vi "Bench Encode PNG.vi"() -> ()   [LabVIEW 2020]
doc: "Benchmark for RemoteVI Capture Panel.vi and RemoteVI Encode Rect PNG.vi. Opens the panel of the VI at VI Path, waits, captures it once (timed), closes the panel and the reference without saving, then encodes the full capture and a 64-row band at every compression level in Levels and reports the average milliseconds and PNG sizes. Writes the full capture, encoded with the default compression, to PNG Path."
uses:
  source/RemoteVI.lvlib
panel:
  out "error out":errorcluster
  out "default png bytes":i32
  out "band bytes":i32[](array[numeric])
  out "band ms":dbl[](array[numeric])
  out "full bytes":i32[](array[numeric])
  out "full ms":dbl[](array[numeric])
  out "capture ms":i32
  out "height":i32
  out "width":i32
  in  "Settle ms":i32=1000
  in  "Band Top":i32=256
  in  "Band Reps":i32=20
  in  "Full Reps":i32=5
  in  "Levels":i32[](array[numeric])=[0, 1, 2, 3, 6, 9]
  in  "PNG Path":path=path "C:/Users/jgoebel/OneDrive - Emerson/Dokumente/git_repos/RemoteVI/spikes/encode_check.png"
  in  "VI Path":path=path "C:/Program Files/National Instruments/LabVIEW 2025/examples/Controls and Indicators/Containers/Resizable Panel with Splitter Bars.vi"
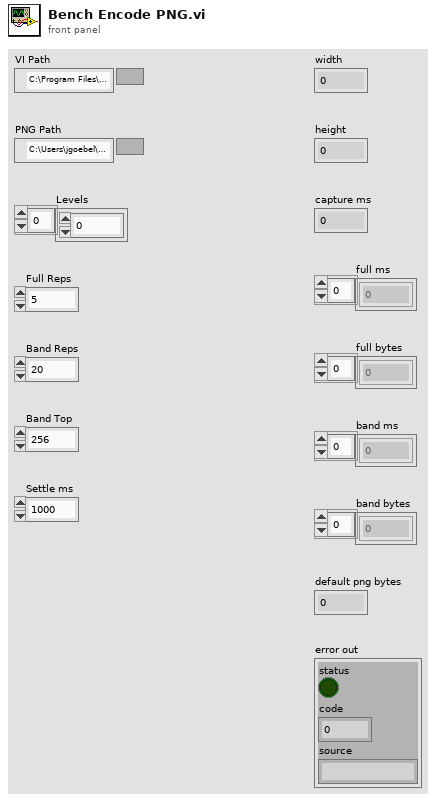
[diagram p1: front panel]
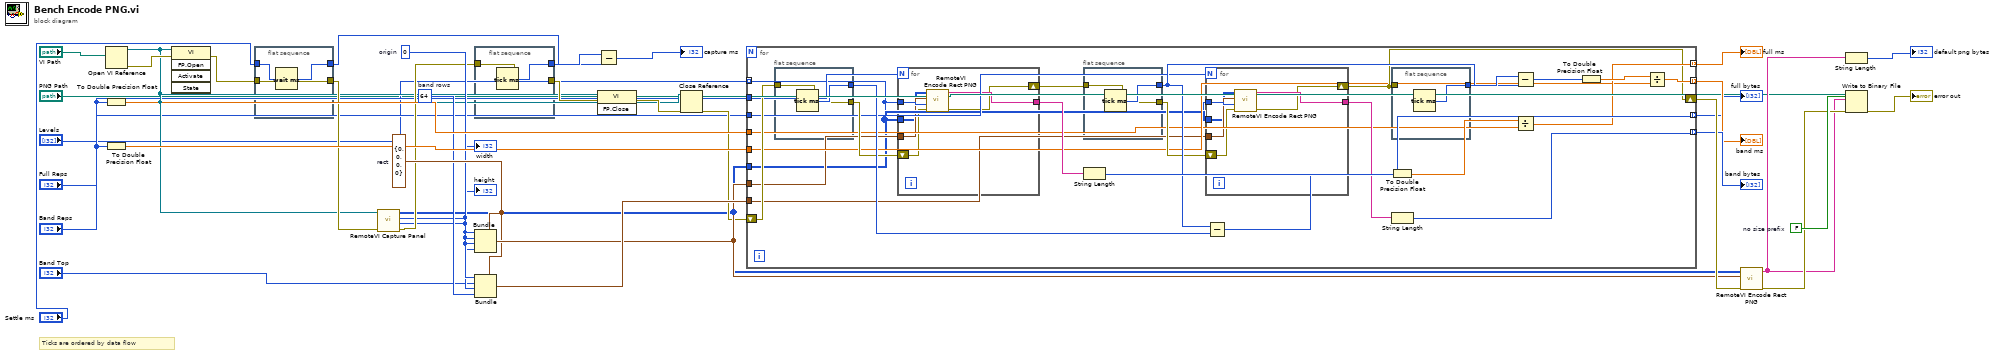
[diagram p0: block diagram]
diagram:
  w38 = FALSE  # no size prefix
  w30 = cluster{"x":i32, "y":i32, "w":i32, "h":i32} {"x"=0, "y"=0, "w"=0, "h"=0}  # rect
  w29 = 64  # band rows
  w28 = 0  # origin
  # "Ticks are ordered by data flow"
  n1 = Open VI Reference(vi path="VI Path") -> (vi reference=w17:refnum<vi>, error out=w18:errorcluster)  [unwired: 5 in]
  n2 = To Double Precision Float(number="Full Reps") -> (double precision float=w33:dbl)
  n3 = To Double Precision Float(number="Band Reps") -> (double precision float=w34:dbl)
  n4 = invoke class="VI" method="FP.Open"(reference=w17, error in=w18) -> (error out=w19:errorcluster)  [unwired: 3 in, 4 out]
  n5 = flat-sequence {
    tunnel: "Settle ms" -> [w40]
    tunnel: w19 -> [w39]
    tunnel: [w41] -> w21
    tunnel: [w39] -> w20
    frame #0 {
      n6 = Wait (ms)(milliseconds to wait=w40) -> (millisecond timer value=w41:i32)
    }
  }
  n7 = call "RemoteVI Capture Panel.vi"("error in"=w20, "VI"=w17) -> ("error out"=w23:errorcluster, "height"=w9:i32, "width"=w8:i32, "pixmap"=w22:u32[][])  [unwired: 6 in]
  "width" <- w8
  "height" <- w9
  n8 = flat-sequence {
    tunnel: [w43] -> w25
    tunnel: w23 -> [w42]
    tunnel: [w42] -> w24
    frame #0 {
      n9 = Tick Count (ms)() -> (millisecond timer value=w43:u32)
    }
  }
  n10 = Bundle(cluster=w30, "x"=w28, "y"=w28, "w"=w8, "h"=w9) -> (w31:cluster{"x":i32, "y":i32, "w":i32, "h":i32})
  n11 = Bundle(cluster=w30, "x"=w28, "y"="Band Top", "w"=w8, "h"=w29) -> (w32:cluster{"x":i32, "y":i32, "w":i32, "h":i32})
  n12 = Subtract(x=w25, y=w21) -> (x-y=→"capture ms":u32)
  n13 = invoke class="VI" method="FP.Close"(reference=w17, error in=w24) -> (error out=w26:errorcluster)  [unwired: 1 in, 2 out]
  n14 = Close Reference(reference=w17, error in (no error)=w26) -> (error out=w27:errorcluster)
  n15 = for {
    tunnel: "Levels" -> [w44] mode=indexing
    tunnel: "Full Reps" -> [w48]
    tunnel: "Band Reps" -> [w49]
    tunnel: w33 -> [w50]
    tunnel: w34 -> [w51]
    tunnel: w22 -> [w45]
    tunnel: [w64] -> w11 mode=indexing
    tunnel: [w67] -> w13 mode=indexing
    tunnel: w31 -> [w46]
    tunnel: w32 -> [w47]
    shift-right: [w53] -> w35
    shift-left: w27 -> [w52]
    tunnel: [w68] -> w12 mode=indexing
    tunnel: [w69] -> w14 mode=indexing
    n16 = flat-sequence {
      tunnel: [w86] -> w55
      tunnel: w52 -> [w85]
      tunnel: [w85] -> w54
      frame #0 {
        n17 = Tick Count (ms)() -> (millisecond timer value=w86:u32)
      }
    }
    n18 = for {
      N: w48 -> [_]
      tunnel: w44 -> [w81]
      tunnel: w45 -> [w79]
      tunnel: w46 -> [w80]
      shift-right: [w83] -> w56
      shift-left: w54 -> [w82]
      tunnel: [w84] -> w57
      n19 = call "RemoteVI Encode Rect PNG.vi"("error in"=w82, "compression"=w81, "rect"=w80, "pixmap"=w79) -> ("error out"=w83:errorcluster, "png"=w84:string)  [unwired: 6 in]
    }
    n20 = flat-sequence {
      tunnel: [w78] -> w59
      tunnel: w56 -> [w77]
      tunnel: [w77] -> w58
      frame #0 {
        n21 = Tick Count (ms)() -> (millisecond timer value=w78:u32)
      }
    }
    n22 = String Length(string=w57) -> (length=w68:i32)
    n23 = for {
      N: w49 -> [_]
      tunnel: w44 -> [w73]
      tunnel: w45 -> [w71]
      tunnel: w47 -> [w72]
      shift-right: [w75] -> w53
      shift-left: w58 -> [w74]
      tunnel: [w76] -> w60
      n24 = call "RemoteVI Encode Rect PNG.vi"("error in"=w74, "compression"=w73, "rect"=w72, "pixmap"=w71) -> ("error out"=w75:errorcluster, "png"=w76:string)  [unwired: 6 in]
    }
    n25 = Subtract(x=w59, y=w55) -> (x-y=w62:u32)
    n26 = flat-sequence {
      tunnel: [w70] -> w61
      tunnel: w53 -> [_]
      frame #0 {
        n27 = Tick Count (ms)() -> (millisecond timer value=w70:u32)
      }
    }
    n28 = To Double Precision Float(number=w62) -> (double precision float=w63:dbl)
    n29 = String Length(string=w60) -> (length=w69:i32)
    n30 = Subtract(x=w61, y=w59) -> (x-y=w65:u32)
    n31 = Divide(x=w63, y=w50) -> (x/y=w64:dbl)
    n32 = To Double Precision Float(number=w65) -> (double precision float=w66:dbl)
    n33 = Divide(x=w66, y=w51) -> (x/y=w67:dbl)
  }
  "full ms" <- w11
  "full bytes" <- w12
  "band ms" <- w13
  "band bytes" <- w14
  n34 = call "RemoteVI Encode Rect PNG.vi"("error in"=w35, "rect"=w31, "pixmap"=w22) -> ("error out"=w37:errorcluster, "png"=w36:string)  [unwired: 7 in]
  n35 = String Length(string=w36) -> (length=→"default png bytes":i32)
  n36 = Write to Binary File(file (use dialog)="PNG Path", data=w36, error in=w37, 5:w38) -> (error out=→"error out":errorcluster)  [unwired: 2 in, 2 out]
